vi "suhas&claire-encoder_motor&y.vi"() -> ()   [LabVIEW 2026]
uses:
  <vilib>/DAQmx/read.llb/DAQmx Read (Counter DBL 1Chan 1Samp).vi
  <vilib>/Utility/file.llb/Write Delimited Spreadsheet (string).vi
panel:
  out "Y Velocity (mm/s)":dbl
  out "Y Position (mm)":dbl
  out "Invert X":bool
  in  "Motor Clock Num per Pulse":u32=100
  in  "Port0 Bits 2":tag="Dev1/port0/line0:7"
  in  "Laser Sync Source":tag="/Dev1/PFI8"
  in  "Laser DO Rate":u32=40000
  in  "Motor Pulse Rate 2":i32=200
  in  "kx":dbl=1.0
  in  "Move X 2":bool
  in  "delta_x 2":dbl=1.0
  in  "xdir 2":bool=TRUE
  out "Time Between Pulse":dbl
  in  "stop":bool
  out "Logging":bool
  out "Saving to":path
  out "XY Graph":cluster{i16[], dbl[]}(graph)
  out "Pulse Count":dbl
  out "X Velocity (mm/s)":dbl
  out "X Position (mm)":dbl
  # "mm"
  # "mm/s"
  # "(steps/mm)"
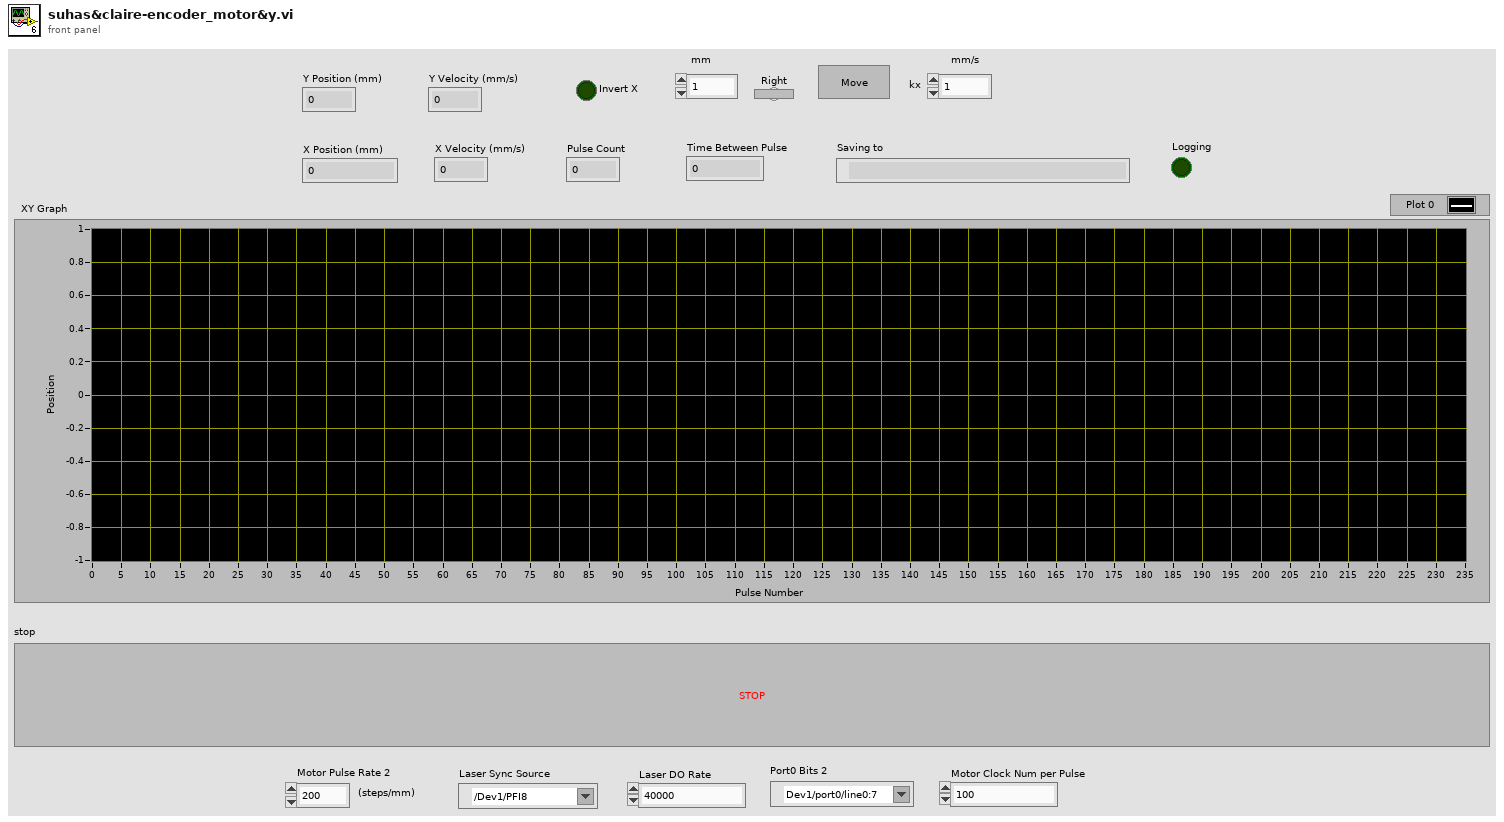
[diagram p1: front panel]
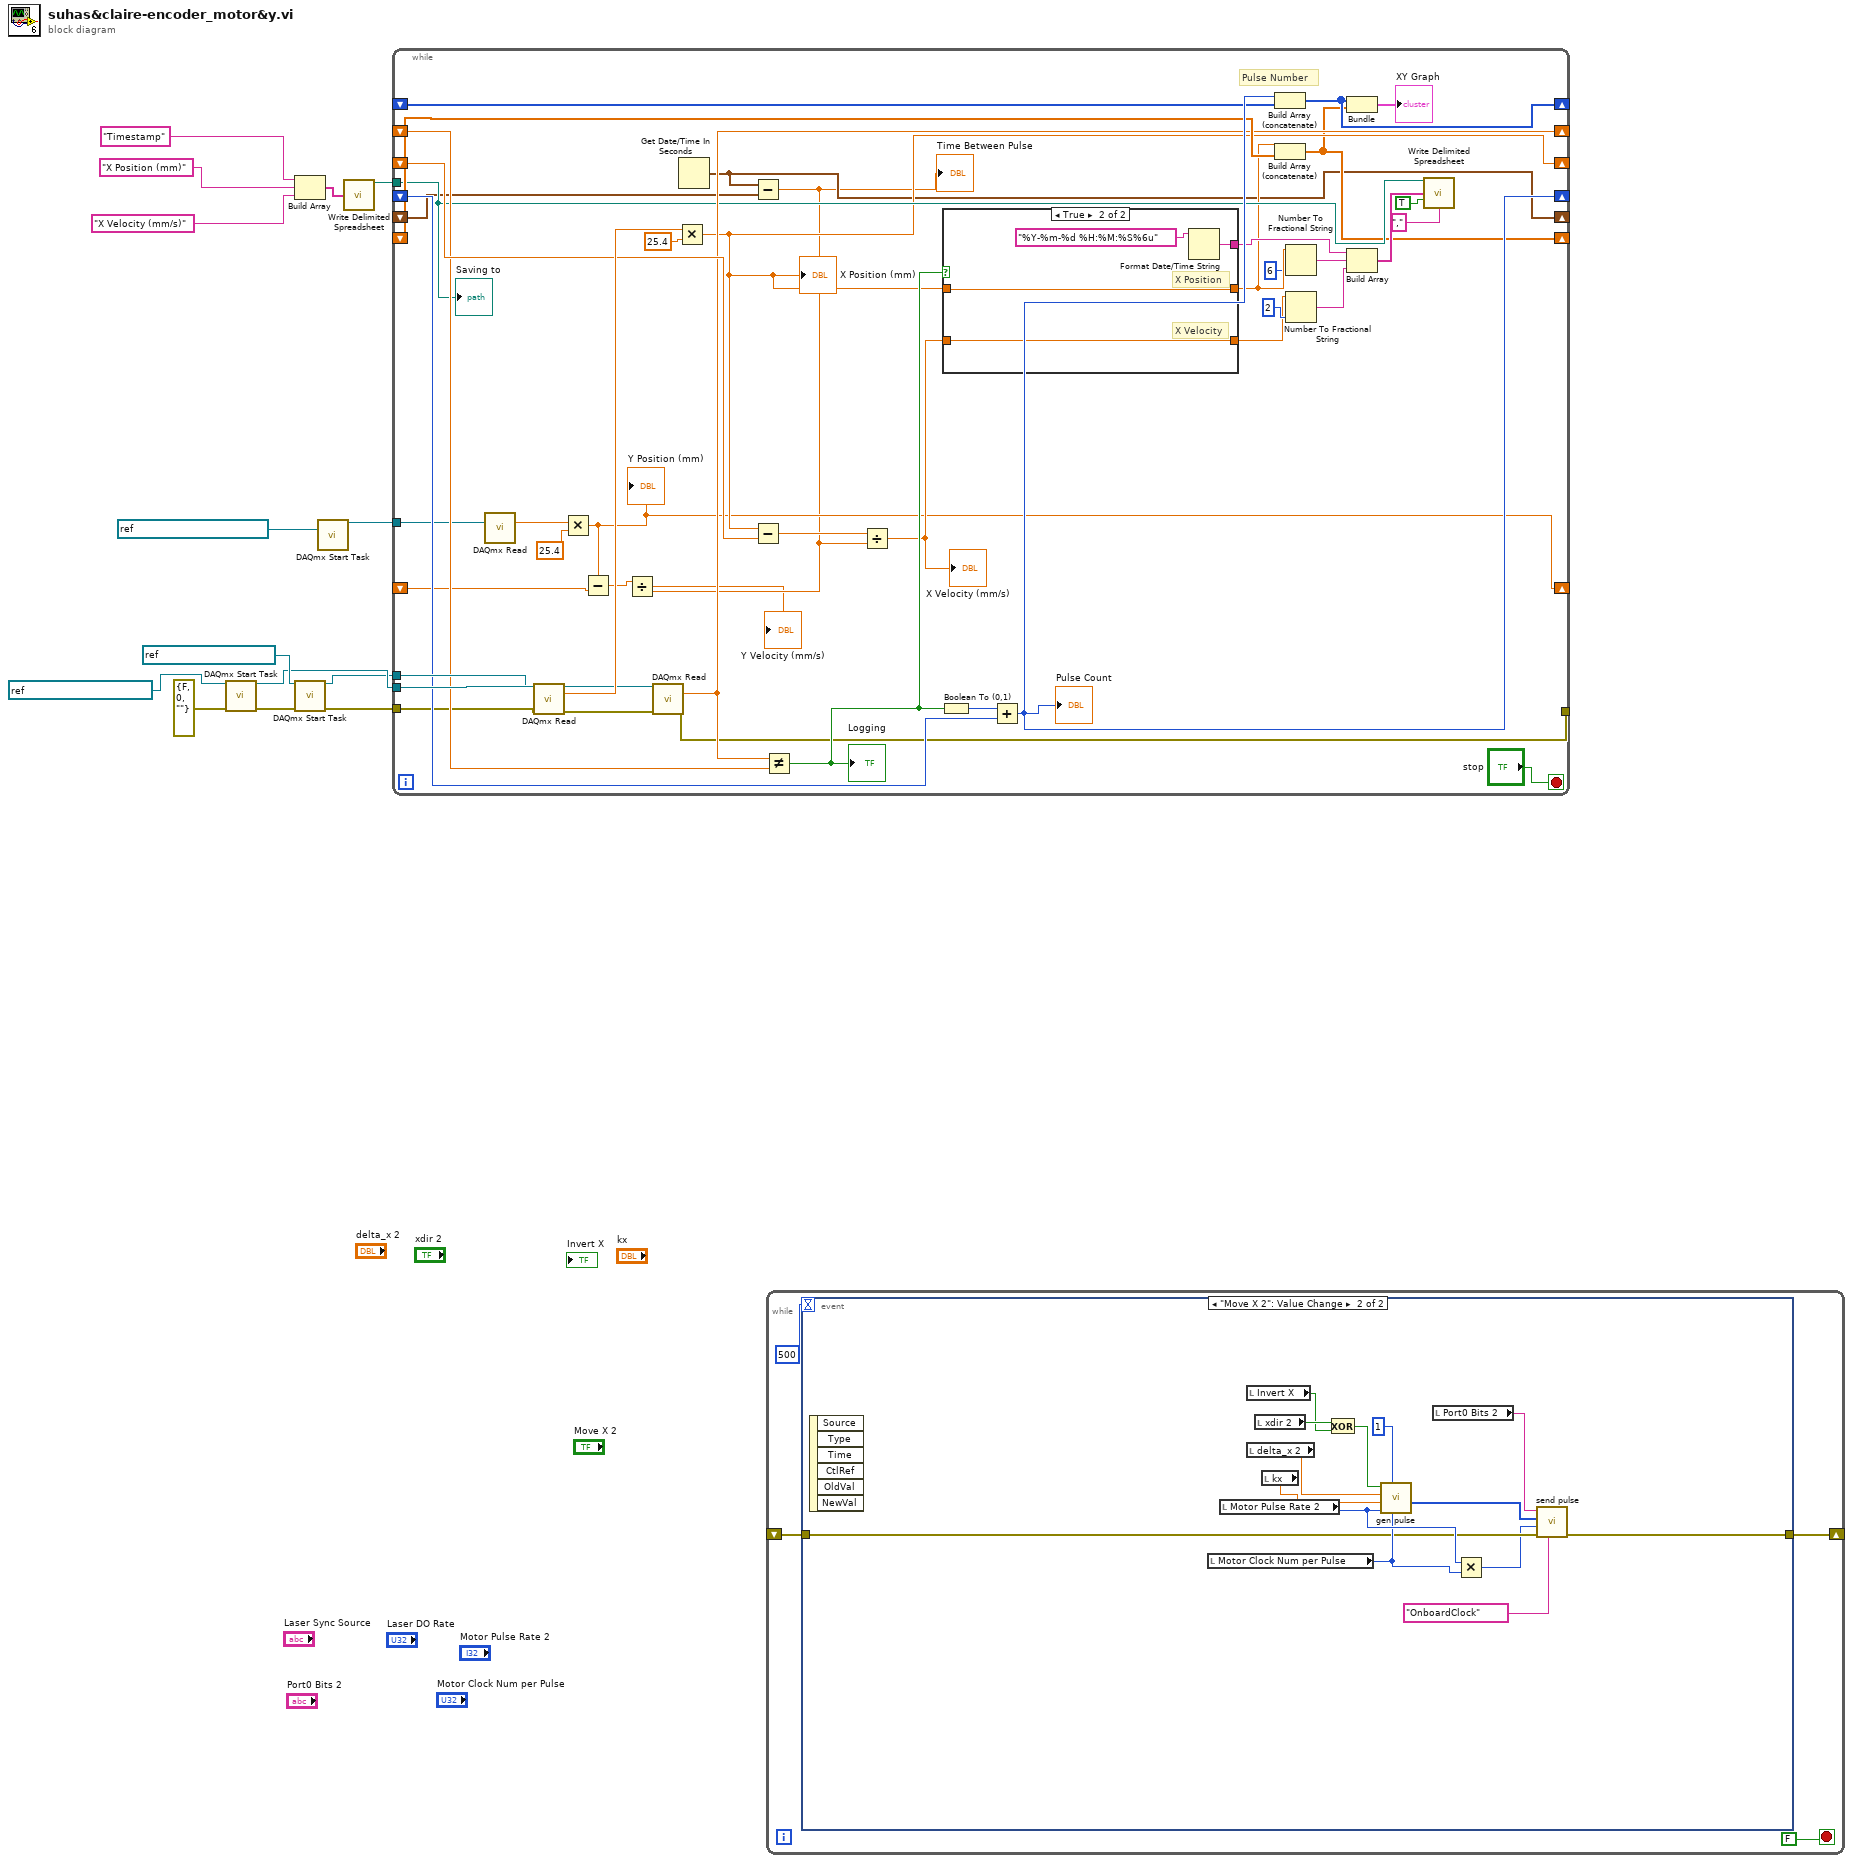
[diagram p0: block diagram]
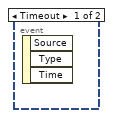
[diagram p2: hidden frame]
diagram:
  n1 = call <vilib>:"DAQmx Start Task.vi"("task/channels in"=refnum<k21> "MyLinearPositionTask", "error in"=errorcluster {"status"=FALSE, "code"=0, "source"=""}) -> ("task out"=w11:refnum<k21>, "error out"=w5:errorcluster)  [unwired: 12 in]
  n2 = Build Array("Timestamp", "X Position (mm)", "X Velocity (mm/s)") -> (w7:string[])
  n3 = call <vilib>:"DAQmx Start Task.vi"("task/channels in"=refnum<k21> "MyCountEdgesTask", "error in"=w5) -> ("task out"=w10:refnum<k21>, "error out"=w4:errorcluster)  [unwired: 12 in]
  n4 = call <vilib>:"DAQmx Start Task.vi"("task/channels in"=refnum<k21> "MyLinearPositionTaskY") -> ("task out"=w1:refnum<k21>)  [unwired: 13 in, 1 out]
  n5 = call-poly <vilib>:"Write Delimited Spreadsheet.vi"("1D data"=w7) -> ("new file path (Not A Path if cancelled)"=w6:path)  [unwired: 13 in, 1 out]
  n6 = while {
    tunnel: w11 -> [w57]
    tunnel: w10 -> [w54]
    shift-right: [w44] -> _
    shift-left: _ -> [w43]
    shift-right: [w33] -> _
    shift-left: _ -> [w52]
    shift-right: [w48] -> _
    shift-left: _ -> [w49]
    shift-right: [w42] -> _
    shift-left: _ -> [w47]
    shift-right: [w27] -> _
    shift-left: _ -> [w46]
    tunnel: w6 -> [w35]
    shift-right: [w24] -> _
    shift-left: _ -> [w34]
    tunnel: w4 -> [w29]
    tunnel: [w28] -> _
    tunnel: w1 -> [w22]
    shift-right: [w18] -> _
    shift-left: _ -> [w19]
    stop <- "stop" stop-if-true
    # "Pulse Number"
    n7 = call-poly <vilib>:"DAQmx Read.vi"("task/channels in"=w22) -> ("data"=w21:dbl)  [unwired: 12 in, 2 out]
    n8 = call-poly <vilib>:"DAQmx Read.vi"("task/channels in"=w57, "error in"=w29) -> ("data"=w56:dbl, "error out"=w53:errorcluster)  [unwired: 11 in, 1 out]
    n9 = Multiply(x=w21, y=25.4) -> (x*y=w18:dbl)
    "Y Position (mm)" <- w18
    n10 = Subtract(x=w18, y=w19) -> (x-y=w17:dbl)
    n11 = call-poly <vilib>:"DAQmx Read.vi"("task/channels in"=w54, "error in"=w53) -> ("data"=w44:dbl, "error out"=w28:errorcluster)  [unwired: 11 in, 1 out]
    n12 = Multiply(x=w56, y=25.4) -> (x*y=w33:dbl)
    "X Position (mm)" <- w33
    n13 = Get Date/Time In Seconds() -> (seconds since 1Jan1904=w24:timestamp)
    n14 = Subtract(x=w24, y=w34) -> (x-y=w16:dbl)
    "Time Between Pulse" <- w16
    n15 = Divide(x=w17, y=w16) -> (x/y=→"Y Velocity (mm/s)":dbl)
    n16 = Subtract(x=w33, y=w52) -> (x-y=w51:dbl)
    n17 = Not Equal?(x=w44, y=w43) -> (x != y?=w45:bool)
    "Logging" <- w45
    n18 = Divide(x=w51, y=w16) -> (x/y=w32:dbl)
    "X Velocity (mm/s)" <- w32
    n19 = Boolean To (0,1)(Boolean=w45) -> (0, 1=w50:i16)
    n20 = case shown="True" w45 {
      tunnel: [_ w61] -> w40
      tunnel: w33 -> [_ w60]
      tunnel: [_ w60] -> w30
      tunnel: w32 -> [_ w59]
      tunnel: [_ w59] -> w31
      frame False {
      }
      frame True {
        # "X Velocity"
        # "X Position"
        n21 = Format Date/Time String(time format string (%c)="%Y-%m-%d %H:%M:%S%6u") -> (date/time string=w61:string)  [unwired: 2 in]
      }
    }
    n22 = Add(x=w50, y=w49) -> (x+y=w48:i16)
    "Pulse Count" <- w48
    n23 = Build Array (concatenate)(w48, w47) -> (w42:i16[])
    n24 = Build Array (concatenate)(w30, w46) -> (w27:dbl[])
    n25 = Number To Fractional String(number=w30, precision (6)=i16 6) -> (F-format string=w39:string)  [unwired: 2 in]
    n26 = Number To Fractional String(number=w31, precision (6)=i16 2) -> (F-format string=w25:string)  [unwired: 2 in]
    n27 = Bundle(w42, w27) -> (→"XY Graph":cluster{i16[], dbl[]})  [unwired: 1 in]
    n28 = Build Array(w40, w39, w25) -> (w38:string[])
    n29 = call-poly <vilib>:"Write Delimited Spreadsheet.vi"("file path (dialog if empty)"=w35, "1D data"=w38, "append to file? (new file:F)"=TRUE, "delimiter (\\t)"="," ("delimiter (\\t)")) -> ()  [unwired: 10 in, 2 out]
    "Saving to" <- w35
  }
  n30 = while {
    shift-right: [w65] -> _
    shift-left: _ -> [w64]
    stop <- FALSE stop-if-true
    n31 = event shown="[1] \"Move X 2\": Value Change" {
      selector: _ -> [_ _]
      dyn-events: _ -> [_ _]
      timeout: 500 -> [_ _]
      tunnel: [_ w68] -> w65
      tunnel: w64 -> [_ w72]
      event Timeout {
        n32 = event-data() -> ()  [unwired: 1 in, 3 out]
      }
      event "Move X 2": Value Change {
        n33 = event-data() -> ()  [unwired: 1 in, 6 out]
        n34 = local read "Motor Clock Num per Pulse"() -> (w73:u32)
        n35 = local read "Motor Pulse Rate 2"() -> (w74:i32)
        n36 = local read "Invert X"() -> (w79:bool)
        n37 = local read "delta_x 2"() -> (w76:dbl)
        n38 = local read "xdir 2"() -> (w80:bool)
        n39 = local read "kx"() -> (w75:dbl)
        n40 = Exclusive Or(1:w79, 2:w80) -> (0:w77:bool)
        n41 = call "gen pulse.vi"("clk per pulse"=w73, "bit"=u8 1, "Motor Pulse Rate / mm"=w74, "kx"=w75, "xn"=w76, "dir"=w77) -> ("pulsetrain"=w70:u8[])  [unwired: 3 in, 2 out]
        n42 = local read "Port0 Bits 2"() -> (w71:tag)
        n43 = Multiply(x=w74, y=w73) -> (x*y=w69:u32)
        n44 = call "send pulse.vi"("source"=tag "OnboardClock", "error in"=w72, "Motors DO rate"=w69, "P0 DO data"=w70, "Port0 Bits"=w71) -> ("error out"=w68:errorcluster)  [unwired: 6 in]
      }
    }
  }
